vi "CANsub_Echo_API.vi"() -> ()   [LabVIEW 2021]
doc: "S5 echo through the CANsub API (A5b): Init/Frames_Create/Open, loop {Read ? Echo_Handle_Frames_API (Write_Echo, UDP reports)}, Status, Close. Reference for the A6 A/B runs against CANsub_Echo_C."
uses:
  api/CANsub_Channel/CANsub_Channel.lvclass
  Echo_Context.ctl
  Echo_Time_Store.ctl
  Echo_Counters.ctl
  common/Typedefs/CANsub_connection.ctl
  common/CANsub_Common.lvlib
  common/Typedefs/CANsub_Bit_Rates.ctl
  api/Typedefs/CANsub_Filter.ctl
  api/CANsub_API.lvlib
  api/Typedefs/CANsub_Read_Mode.ctl
  api/Typedefs/CANsub_Ownership.ctl
  api/Typedefs/CANsub_Config.ctl
  Echo_Config.ctl
  api/Typedefs/CANsub_State.ctl
  common/Typedefs/Bit_Timing.ctl
  api/Typedefs/CANsub_Status.ctl
panel:
  out "error out":errorcluster
  out "status":T1
  out "counters":T4
  in  "stop":bool
  in  "echo config":T5={"echo offset"=-256, "base id"=256, "report port"=5302} {"base id" format="%.0x"}
  in  "config":T6={"connection"={"host"="192.168.0.49", "channel"=2, "cert path"=path "/home/lvuser/cansub_root_cert.crt"}, "bit rates"={"nominal bit rate"=500000, "nominal sample point"=80.0, "data bit rate"=2000000, "data sample point"=80.0}, "listen only"=FALSE, "filters"=[], "read mode"=enum."Poll", "max bytes per read"=4096, "reader FIFO depth"=0, "reader priority"=0, "ownership"=enum."Direct"} {"filters"."f2" format="%.0x"; "filters"."f1" format="%.0x"}
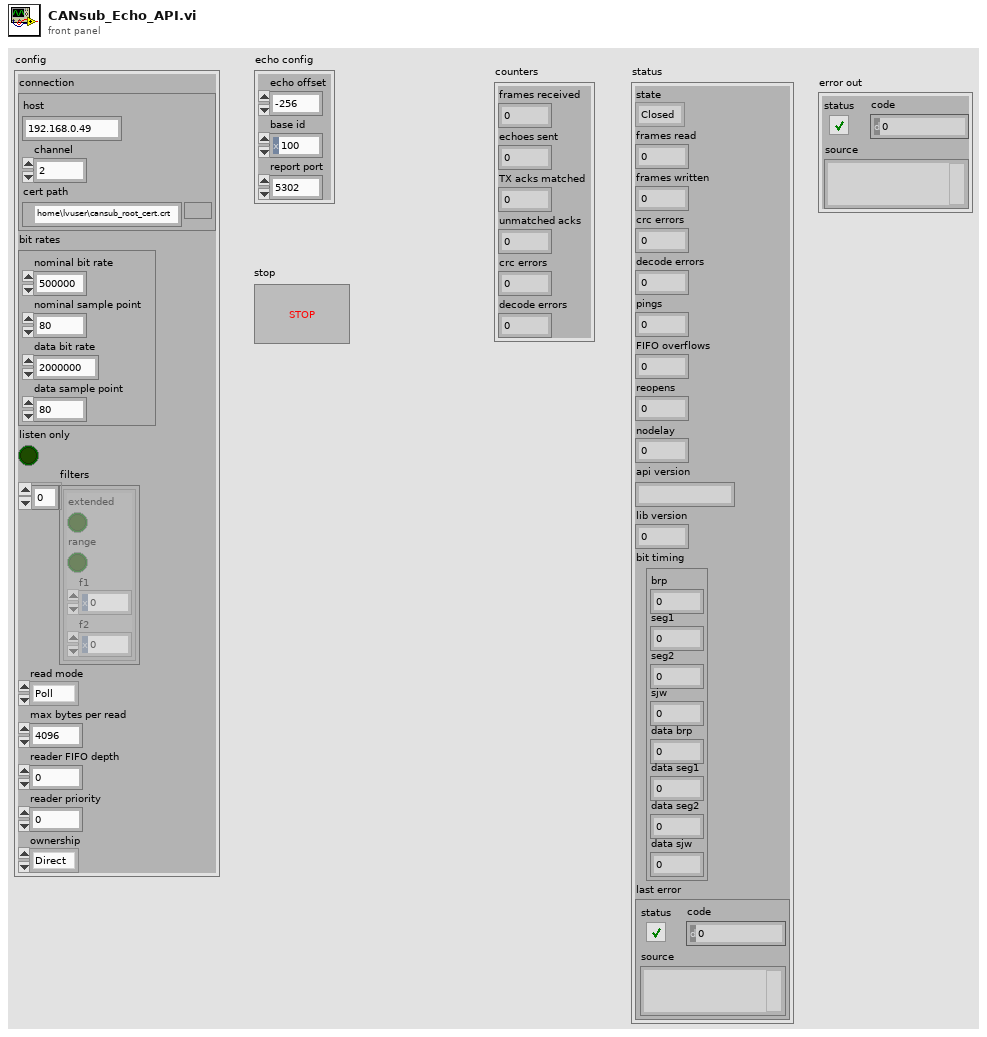
[diagram p1: front panel]
types:
  T1 = typedef "CANsub_API.lvlib/CANsub_Status.ctl" = cluster{"state":T2, "frames read":u32, "frames written":u32, "crc errors":u32, "decode errors":i32, "pings":u32, "FIFO overflows":u32, "reopens":u32, "nodelay":i32, "api version":string, "lib version":u32, "bit timing":T3, "last error":errorcluster}
  T2 = typedef "CANsub_API.lvlib/CANsub_State.ctl" = enum16{"Closed", "Open", "Lost"}
  T3 = typedef "CANsub_Common.lvlib/Bit_Timing.ctl" = cluster{"brp":u16, "seg1":u16, "seg2":u16, "sjw":u16, "data brp":u16, "data seg1":u16, "data seg2":u16, "data sjw":u16}
  T4 = typedef "Echo_Counters.ctl" = cluster{"frames received":u32, "echoes sent":u32, "TX acks matched":u32, "unmatched acks":u32, "crc errors":u32, "decode errors":i32}
  T5 = typedef "Echo_Config.ctl" = cluster{"echo offset":i32, "base id":u32, "report port":u16}
  T6 = typedef "CANsub_API.lvlib/CANsub_Config.ctl" = cluster{"connection":T7, "bit rates":T8, "listen only":bool, "filters":T9[], "read mode":T10, "max bytes per read":i32, "reader FIFO depth":i32, "reader priority":i32, "ownership":T11}
  T7 = typedef "CANsub_Common.lvlib/CANsub_connection.ctl" = cluster{"host":string, "channel":u8, "cert path":path}
  T8 = typedef "CANsub_Common.lvlib/CANsub_Bit_Rates.ctl" = cluster{"nominal bit rate":u32, "nominal sample point":dbl, "data bit rate":u32, "data sample point":dbl}
  T9 = typedef "CANsub_API.lvlib/CANsub_Filter.ctl" = cluster{"extended":bool, "range":bool, "f1":u32, "f2":u32}
  T10 = typedef "CANsub_API.lvlib/CANsub_Read_Mode.ctl" = enum16{"Poll", "Reader"}
  T11 = typedef "CANsub_API.lvlib/CANsub_Ownership.ctl" = enum16{"Direct", "Shared"}
  T12 = typedef "Echo_Time_Store.ctl" = cluster{"t_rx2_dev":dbl[], "t_rx2_lv":dbl[], "t_echo_send_lv":dbl[]}
  T13 = typedef "Echo_Context.ctl" = cluster{"TLS connection":refnum<k5>, "udp":refnum<k16>, "lv addr":u32, "report port":u16, "test lo":u32, "test hi":u32, "ack lo":u32, "ack hi":u32, "echo offset":i32}
  T14 = typedef "CANsub_API.lvlib/CANsub_Frames.ctl" = cluster{"count":i32, "t_dev":dbl[], "id":u32[], "flags":u16[], "dlc":u8[], "data len":u8[], "data":u8[]}
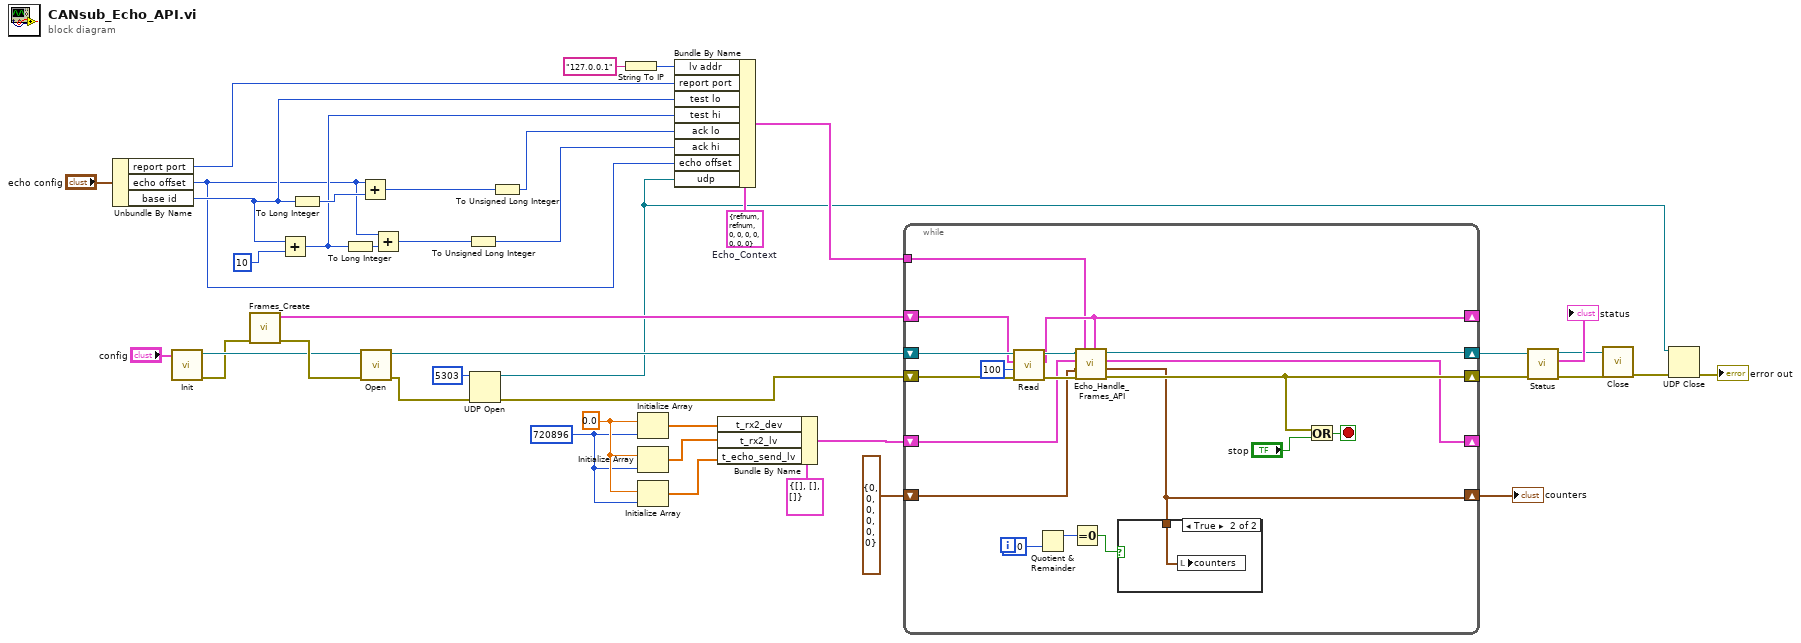
[diagram p0: block diagram]
diagram:
  w26 = 720896 ("dimension size")
  w27 = 0.0
  w36 = T13 {"TLS connection"=refnum, "udp"=refnum, "lv addr"=0, "report port"=0, "test lo"=0, "test hi"=0, "ack lo"=0, "ack hi"=0, "echo offset"=0}  # Echo_Context
  n1 = Unbundle By Name("echo config") -> ("report port"=w34:u16, "echo offset"=w29:i32, "base id"=w31:u32)
  n2 = call "Init.vi"("config"="config") -> ("error out"=w13:errorcluster, "channel out"=w16:refnum<class "CANsub_Channel.lvclass">)  [unwired: 8 in, 1 out]
  n3 = call "Frames_Create.vi"("error in (no error)"=w13) -> ("error out"=w17:errorcluster, "frames"=w14:T14)  [unwired: 9 in]
  n4 = Add(x=w31, y=u32 10) -> (x+y=w30:u32)
  n5 = To Long Integer(number=w31) -> (32bit integer=w40:i32)
  n6 = To Long Integer(number=w30) -> (32bit integer=w39:i32)
  n7 = Add(x=w29, y=w40) -> (x+y=w38:i32)
  n8 = call-dynamic "Open.vi"("error in (no error)"=w17, "channel in"=w16) -> ("error out"=w12:errorcluster, "channel out"=w15:refnum<class "CANsub_Channel.lvclass">)  [unwired: 8 in]
  n9 = Add(x=w29, y=w39) -> (x+y=w37:i32)
  n10 = To Unsigned Long Integer(number=w37) -> (unsigned 32bit integer=w32:u32)
  n11 = UDP Open(8:w12, 11:u16 5303 ("port")) -> (port=w2:refnum<k16>, 0:w10:errorcluster)  [unwired: 3 in, 1 out]
  n12 = To Unsigned Long Integer(number=w38) -> (unsigned 32bit integer=w33:u32)
  n13 = String To IP(1:"127.0.0.1" ("name")) -> (0:w35:u32)
  n14 = Initialize Array(w27, w26) -> (w24:dbl[])
  n15 = Initialize Array(w27, w26) -> (w23:dbl[])
  n16 = Initialize Array(w27, w26) -> (w22:dbl[])
  n17 = Bundle By Name(cluster=w36, "lv addr"=w35, "report port"=w34, "test lo"=w31, "test hi"=w30, "ack lo"=w33, "ack hi"=w32, "echo offset"=w29, "udp"=w2) -> (w11:T13)
  n18 = Bundle By Name(cluster=T12 {"t_rx2_dev"=[], "t_rx2_lv"=[], "t_echo_send_lv"=[]} ("Echo_Time_Store"), "t_rx2_dev"=w24, "t_rx2_lv"=w23, "t_echo_send_lv"=w22) -> (w19:T12)
  n19 = while {
    shift-right: [w43] -> w1
    shift-left: T4 {"frames received"=0, "echoes sent"=0, "TX acks matched"=0, "unmatched acks"=0, "crc errors"=0, "decode errors"=0} ("counters") -> [w50]
    shift-right: [w48] -> _
    shift-left: w19 -> [w51]
    shift-right: [w55] -> w8
    shift-left: w15 -> [w62]
    shift-right: [w52] -> _
    shift-left: w14 -> [w53]
    tunnel: w11 -> [w49]
    shift-right: [w57] -> w5
    shift-left: w10 -> [w59]
    i -> [w44]
    stop <- w60 stop-if-true
    n20 = call-dynamic "Read.vi"("error in (no error)"=w59, "timeout ms"=100, "frames in"=w53, "channel in"=w62) -> ("error out"=w58:errorcluster, "frames out"=w52:T14, "channel out"=w56:refnum<class "CANsub_Channel.lvclass">)  [unwired: 5 in]
    n21 = Quotient & Remainder(x=w44, y=100) -> (x-y*floor(x/y)=w46:i32)  [unwired: 1 out]
    n22 = Equal To 0?(x=w46) -> (x = 0?=w45:bool)
    n23 = call "Echo_Handle_Frames_API.vi"("frames"=w52, "context"=w49, "error in (no error)"=w58, "counters in"=w50, "time store in"=w51, "channel in"=w56) -> ("error out"=w57:errorcluster, "counters out"=w43:T4, "time store out"=w48:T12, "channel out"=w55:refnum<class "CANsub_Channel.lvclass">)  [unwired: 2 in]
    n24 = case shown="True" w45 {
      tunnel: w43 -> [_ w63]
      frame False {
      }
      frame True {
        n25 = local write "counters"(w63) -> ()
      }
    }
    n26 = Or(x=w57, y="stop") -> (x .or. y?=w60:bool)
  }
  "counters" <- w1
  n27 = call-dynamic "Status.vi"("error in (no error)"=w5, "channel in"=w8) -> ("error out"=w6:errorcluster, "status"=→"status":T1, "channel out"=w7:refnum<class "CANsub_Channel.lvclass">)  [unwired: 7 in]
  n28 = call-dynamic "Close.vi"("error in (no error)"=w6, "channel in"=w7) -> ("error out"=w4:errorcluster)  [unwired: 8 in, 1 out]
  n29 = UDP Close(connection ID=w2, 8:w4) -> (error out=→"error out":errorcluster)  [unwired: 1 out]
